vi "Read One Shot TX.vi"(8 "error in (no error)":errorcluster, 11 "CAN_RW_CORE in":refnum<class "CAN_RW_CORE.lvclass">) -> (0 "error out":errorcluster, 2 "One Shot TX":bool=TRUE, 3 "CAN_RW_CORE out":refnum<class "CAN_RW_CORE.lvclass">)   [LabVIEW 2021, in "CAN_RW_CORE.lvclass"]
uses:
  CAN_RW_CORE.lvclass
  CAN_RW_CORE.lvclass/CAN_RW_CORE.ctl
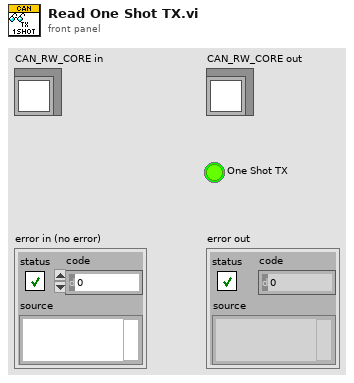
[diagram p1: front panel]
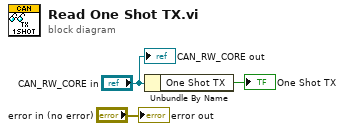
[diagram p0: block diagram]
diagram:
  n1 = Unbundle By Name("CAN_RW_CORE in") -> ("One Shot TX"=→"One Shot TX":bool)
  "error out" <- "error in (no error)"
  "CAN_RW_CORE out" <- "CAN_RW_CORE in"
